vi "ComGlobalVars.vi"() -> ()   [LabVIEW 2026]
uses:
  Typedefs/System_State.ctl
  Typedefs/ServoCommand.ctl
  Typedefs/BeltCtrl.ctl
panel:
  in  "Conveyor Speed":dbl(knob) scale=0.0..10.0
  in  "System State":T1 items=["Idle", "Classify", "Sort"]
  in  "Conveyor Control":T2
  out "Throughput":dbl
  out "Reject bool":bool
  out "Colour 3 bool":bool
  out "Colour 2 bool":bool
  out "Colour 1 bool":bool
  out "Reject":i32
  out "Colour 3":i32
  out "Colour 2":i32
  out "Colour 1":i32
  in  "Servo Control":T3
  out "Auto":bool
  out "Stop System":bool
  out "Live Camera Feed":T4(plugin-control)
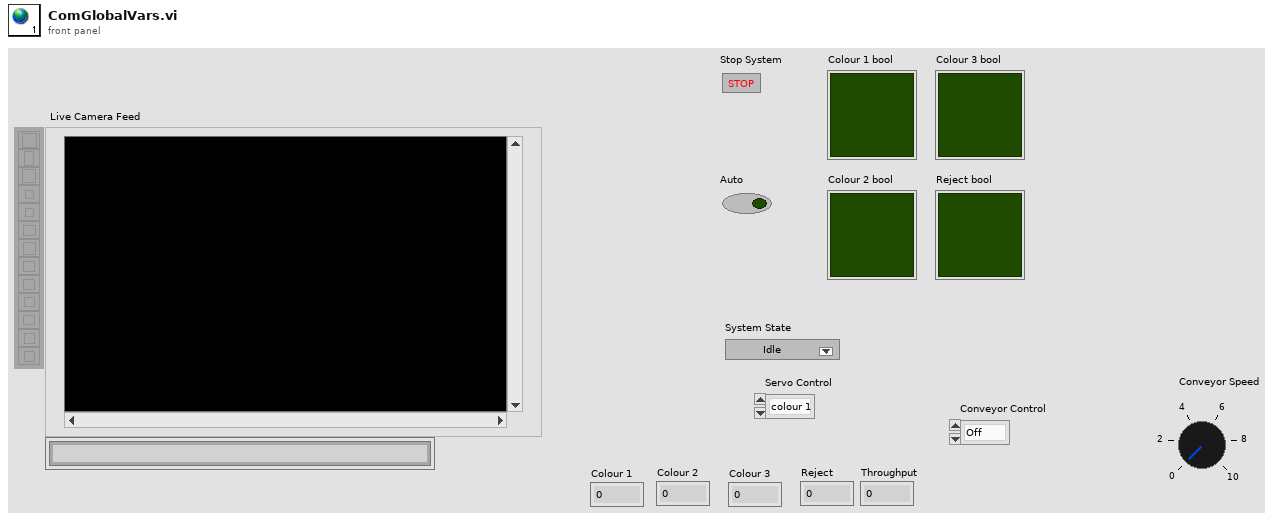
[diagram p1: front panel]
types:
  T1 = typedef "System_State.ctl" = u16
  T2 = typedef "BeltCtrl.ctl" = enum16{"Off", "Forward", "Back", "Coast", "Brake"}
  T3 = typedef "ServoCommand.ctl" = enum16{"colour 1", "Colour2", "Colour3", "Reject"}
  T4 = typedef "IMAQ Image.ctl" = refnum<image>
diagram:
